vi "eDyno Stop and Clear.vi"(0 "AO task":refnum<k21>, 1 "AI task":refnum<k21>, 5 "error in":errorcluster) -> (19 "error out":errorcluster)   [LabVIEW 2026]
doc: "Stops and clears the AO task, then the AI task. Runs even after an upstream error so both tasks are always released."
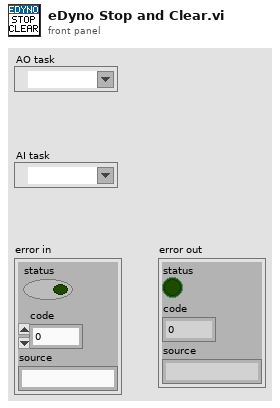
[diagram p1: front panel]
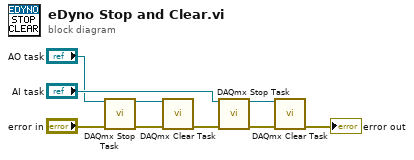
[diagram p0: block diagram]
diagram:
  n1 = call <vilib>:"DAQmx Stop Task.vi"("task/channels in"="AO task", "error in"="error in") -> ("task out"=w5:refnum<k21>, "error out"=w6:errorcluster)  [unwired: 12 in]
  n2 = call <vilib>:"DAQmx Clear Task.vi"("task in"=w5, "error in"=w6) -> ("error out"=w7:errorcluster)  [unwired: 13 in]
  n3 = call <vilib>:"DAQmx Stop Task.vi"("task/channels in"="AI task", "error in"=w7) -> ("task out"=w8:refnum<k21>, "error out"=w9:errorcluster)  [unwired: 12 in]
  n4 = call <vilib>:"DAQmx Clear Task.vi"("task in"=w8, "error in"=w9) -> ("error out"=→"error out":errorcluster)  [unwired: 13 in]
